vi "Read Data from Caller.vi"(7 "lv_icon.vi":refnum<vi>, 8 "error in":errorcluster, 10 "Default body text":T1 {"Body Text Spec"."Alignment" items=["left", "center", "right"]}, 11 "Init? (F)":bool) -> (0 "error out":errorcluster, 1 "Library Icon":picture, 2 "Icon Editor Invoker Type":T5, 3 "data":T4={"Text Visible?"=FALSE, "Text Opacity"=0, "Templ Visible?"=FALSE, "Templ Opacity"=0, "Relative Path from 1 to 2"=path "", "Image"=bytes[0], "All User Layers"=[], "Body Text"={"Line 1 text"="", "Line 2 text"="", "Line 3 text"="", "Line 4 text"="", "Line 1 color"=0, "Line 2 color"=0, "Line 3 color"=0, "Line 4 color"=0, "Body Text Spec"={"Font"="", "Alignment"=0, "Size"=3}, "Center text vertically"=FALSE, "Capitalize Text"=FALSE}} {"Body Text"."Body Text Spec"."Alignment" items=["left", "center", "right"]}, 4 "Valid?":bool, 5 "Valid Library icon?":bool)   [LabVIEW 2020]
uses:
  vi.lib/LabVIEW Icon API/lv_icon/Classes/Layer/Layer.lvclass
  <resource>/plugins/IconEditor/Icon Editor Invoker Type.ctl
  lv_icon.lvlib
  vi.lib/LabVIEW Icon API/lv_icon/Controls/LabVIEW Icon Stored Information.ctl
  vi.lib/LabVIEW Icon API/lv_icon/Controls/Font.ctl
  vi.lib/LabVIEW Icon API/lv_icon/Controls/Alignment.ctl
  vi.lib/LabVIEW Icon API/lv_icon/Controls/BodyText.ctl
panel:
  in  "String":string="Palette Icon"
  in  "Localized string":string="Icon Editor"
  # "Localized Strings"
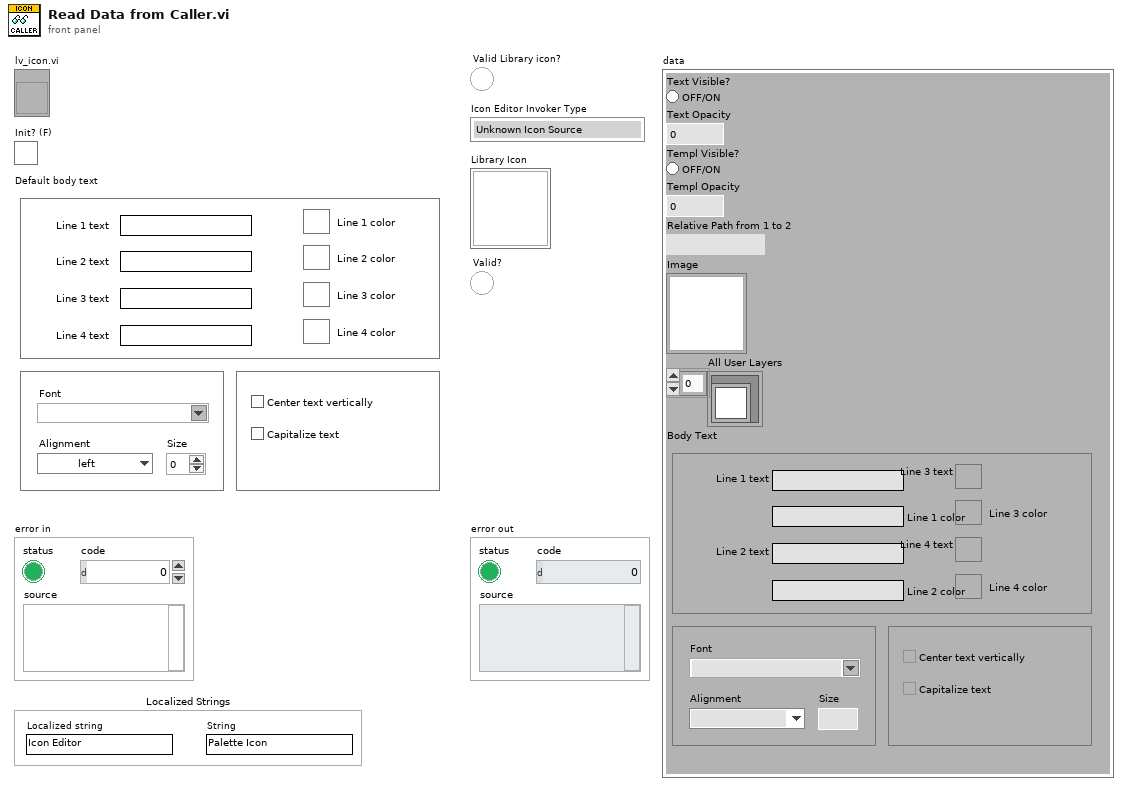
[diagram p1: front panel]
types:
  T1 = typedef "BodyText.ctl" = cluster{"Line 1 text":string, "Line 2 text":string, "Line 3 text":string, "Line 4 text":string, "Line 1 color":u32, "Line 2 color":u32, "Line 3 color":u32, "Line 4 color":u32, "Body Text Spec":cluster{"Font":T2, "Alignment":T3, "Size":u8}, "Center text vertically":bool, "Capitalize Text":bool}
  T2 = typedef "Font.ctl" = string
  T3 = typedef "Alignment.ctl" = u16
  T4 = typedef "LabVIEW Icon Stored Information.ctl" = cluster{"Text Visible?":bool, "Text Opacity":u8, "Templ Visible?":bool, "Templ Opacity":u8, "Relative Path from 1 to 2":path, "Image":picture, "All User Layers":refnum<class "Layer.lvclass">[], "Body Text":T1}
  T5 = typedef "Icon Editor Invoker Type.ctl" = enum32{"Unknown Icon Source", "VI Icon", "Library Icon (any library type)", "Palette icon", "Icon from App Method"}
  T6 = typedef "Who Invoked Icon Editor.ctl" = cluster{"Icon Editor Invoker Type":T5, "App Refnum of Invoker":refnum<vi>, "Qualified Name of Invoker":string, "Path to Invoker":path}
  T7 = typedef "imagedata.ctl" = cluster{"image type":i32, "image depth":i32, "image":u8[], "mask":u8[], "colors":u32[], "Rectangle":cluster{"left":i16, "top":i16, "right":i16, "bottom":i16}}
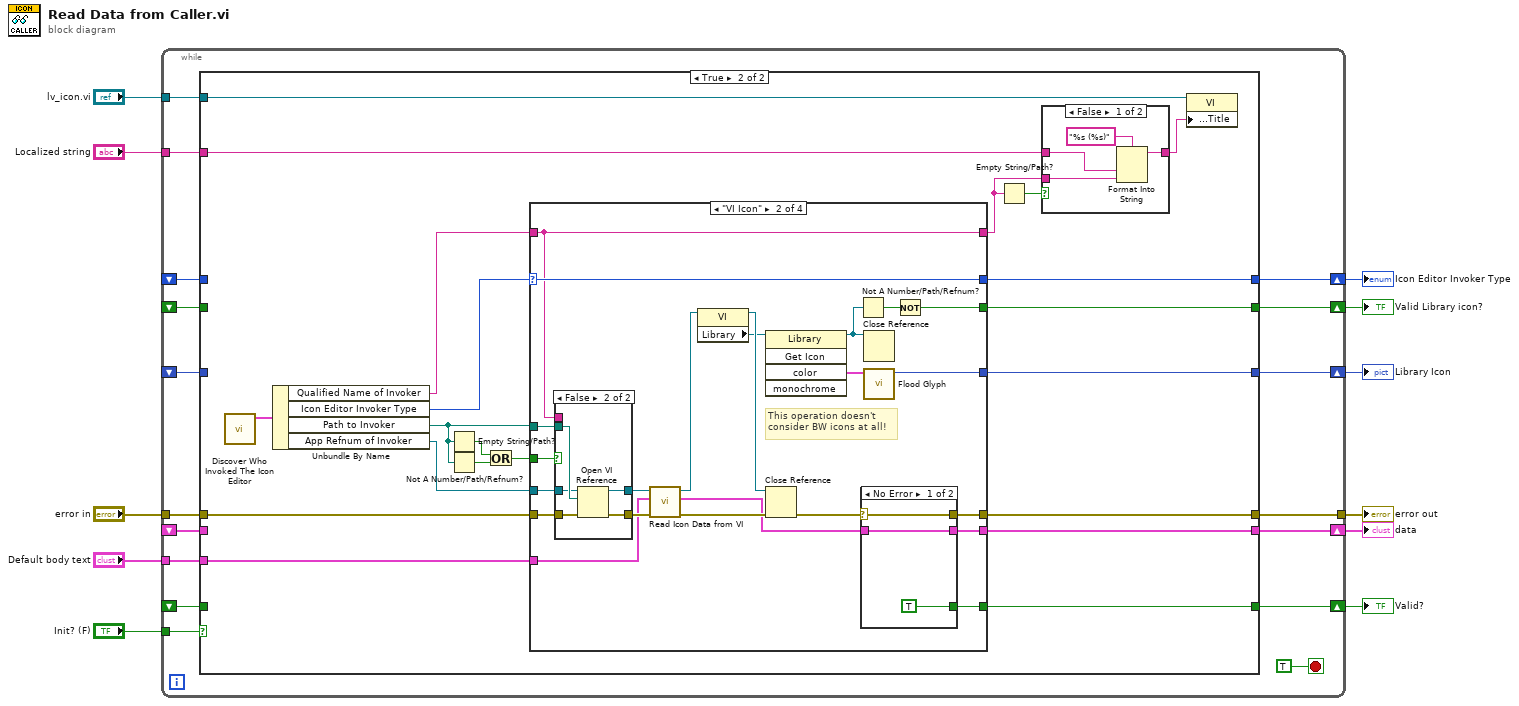
[diagram p0: block diagram]
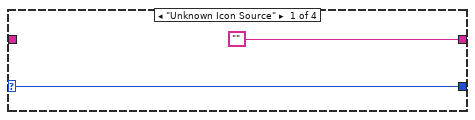
[diagram p4: hidden frame]
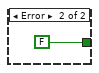
[diagram p5: hidden frame]
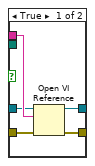
[diagram p6: hidden frame]
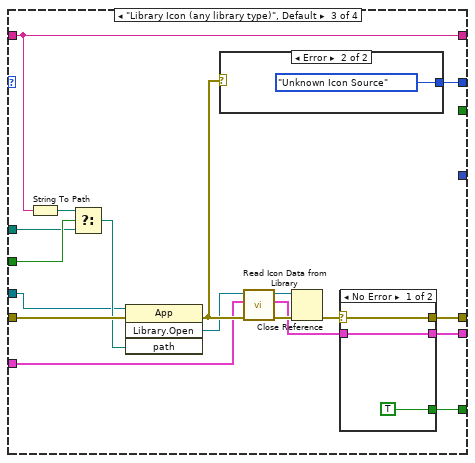
[diagram p7: hidden frame]
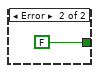
[diagram p8: hidden frame]
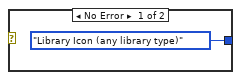
[diagram p9: hidden frame]
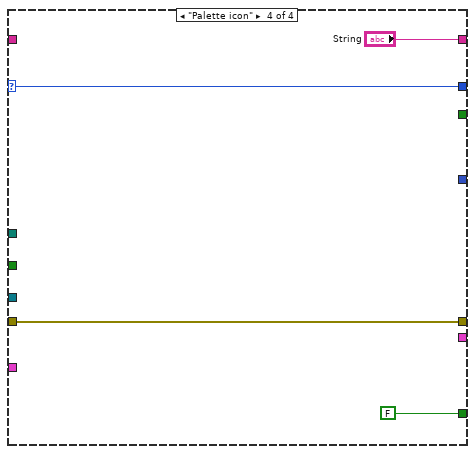
[diagram p10: hidden frame]
diagram:
  n1 = while {
    tunnel: [w28] -> w10
    tunnel: "error in" -> [w27]
    tunnel: "Init? (F)" -> [w24]
    tunnel: "lv_icon.vi" -> [w22]
    shift-right: [w23] -> w7
    shift-left: _ -> [w19]
    shift-right: [w25] -> w5
    shift-left: _ -> [w20]
    shift-right: [w26] -> w6
    shift-left: _ -> [w18]
    shift-right: [w17] -> w4
    shift-left: _ -> [w16]
    shift-right: [w15] -> w3
    shift-left: _ -> [w14]
    tunnel: "Default body text" -> [w13]
    tunnel: "Localized string" -> [w12]
    stop <- TRUE stop-if-true
    n2 = case shown="True" w24 {
      tunnel: [w34 w55] -> w28
      tunnel: [w33 w53] -> w25
      tunnel: [w31 w52] -> w26
      tunnel: w27 -> [w34 w54]
      tunnel: [w32 w48] -> w23
      tunnel: w22 -> [_ w39]
      tunnel: w20 -> [w33 _]
      tunnel: w19 -> [w32 _]
      tunnel: w18 -> [w31 _]
      tunnel: [w30 w42] -> w17
      tunnel: w16 -> [w30 _]
      tunnel: [w29 w35] -> w15
      tunnel: w14 -> [w29 _]
      tunnel: w13 -> [_ w41]
      tunnel: w12 -> [_ w40]
      frame False {
      }
      frame True {
        n3 = call <resource>:"Discover Who Invoked The Icon Editor.vi"() -> ("Who Invoked The Icon Editor?"=w51:T6)  [unwired: 11 out]
        n4 = Unbundle By Name(w51) -> ("Qualified Name of Invoker"=w44:string, "Icon Editor Invoker Type"=w49:T5, "Path to Invoker"=w43:path, "App Refnum of Invoker"=w50:refnum<vi>)
        n5 = Empty String/Path?(string/path=w43) -> (empty?=w47:bool)
        n6 = Not A Number/Path/Refnum?(number/path/refnum=w43) -> (NaN/Path/Refnum?=w46:bool)
        n7 = Or(x=w47, y=w46) -> (x .or. y?=w45:bool)
        n8 = case shown="\"VI Icon\"" w49 {
          selector: w49 -> [w62 w78 _ w125]
          tunnel: [_ w82 w114 w127] -> w55
          tunnel: [_ w65 w100 _] -> w53
          tunnel: [_ w63 w101 FALSE] -> w52
          tunnel: w54 -> [_ w84 w117 w127]
          tunnel: w50 -> [_ w79 w109 _]
          tunnel: [w62 w78 w108 w125] -> w48
          tunnel: w44 -> [_ w66 w103 _]
          tunnel: w43 -> [_ w76 w106 _]
          tunnel: w45 -> [_ w77 w107 _]
          tunnel: [_ w71 _ _] -> w42
          tunnel: [_ w68 _ _] -> w35
          tunnel: w41 -> [_ w67 w104 _]
          tunnel: ["" w66 w103 "String"] -> w36
          frame "Unknown Icon Source" {
          }
          frame "VI Icon" {
            # "This operation doesn't\nconsider BW icons at all!"
            n9 = case shown="False" w77 {
              tunnel: [w92 w96] -> w80
              tunnel: [w94 w99] -> w85
              tunnel: w84 -> [w93 w98]
              tunnel: w79 -> [w90 w95]
              tunnel: w66 -> [w91 _]
              tunnel: w76 -> [_ w97]
              frame True {
                n10 = Open VI Reference(application reference (local)=w90, vi path=w91, error in (no error)=w93) -> (vi reference=w92:refnum<vi>, error out=w94:errorcluster)  [unwired: 3 out]
              }
              frame False {
                n11 = Open VI Reference(application reference (local)=w95, vi path=w97, error in (no error)=w98) -> (vi reference=w96:refnum<vi>, error out=w99:errorcluster)  [unwired: 3 out]
              }
            }
            n12 = call "Read Icon Data from VI.vi"("error in (no error)"=w85, "Default body text"=w67, "VI Ref in"=w80) -> ("error out"=w83:errorcluster, "Data"=w64:T4, "VI Ref out"=w74:refnum<vi>)  [unwired: 6 in]
            n13 = property class="VI"(reference=w74) -> (reference out=w75:refnum<vi>, "Library"=w73:refnum<vi>)  [unwired: 1 in, 1 out]
            n14 = invoke class="Library" method="Get Icon"(reference=w73) -> (reference out=w70:refnum<vi>, "color"=w72:T7)  [unwired: 4 in, 3 out]
            n15 = Close Reference(reference=w75, error in (no error)=w83) -> (error out=w81:errorcluster)
            n16 = Not A Number/Path/Refnum?(number/path/refnum=w70) -> (NaN/Path/Refnum?=w69:bool)
            n17 = case shown="No Error" w81 {
              selector: w81 -> [w88 _]
              tunnel: [w88 _] -> w82
              tunnel: [w86 _] -> w65
              tunnel: [TRUE FALSE] -> w63
              tunnel: w64 -> [w86 _]
              frame No Error {
              }
              frame Error {
              }
            }
            n18 = Close Reference(reference=w70) -> ()  [unwired: 1 in, 1 out]
            n19 = call "Flood Glyph.vi"("image data"=w72) -> ("Pic Out"=w71:picture)  [unwired: 1 in, 9 out]
            n20 = Not(x=w69) -> (.not. x?=w68:bool)
          }
          frame "Library Icon (any library type)", Default {
            n21 = String To Path(string=w103) -> (path=w105:path)
            n22 = Select(t=w105, s=w107, f=w106) -> (s? t:f=w112:path)
            n23 = invoke class="App" method="Library.Open"(reference=w109, error in=w117, "path"=w112) -> (error out=w115:errorcluster, "Open Library"=w111:refnum<vi>)  [unwired: 1 in, 2 out]
            n24 = case shown="Error" w115 {
              tunnel: [Icon_Editor_Invoker_Type."Library Icon (any library type)" ("Icon Editor Invoker Type") Icon_Editor_Invoker_Type."Unknown Icon Source" ("Icon Editor Invoker Type")] -> w108
              frame No Error {
              }
              frame Error {
              }
            }
            n25 = call "Read Icon Data from Library.vi"("error in"=w115, "Default body text"=w104, "Library in"=w111) -> ("error out"=w116:errorcluster, "Data"=w102:T4, "Library out"=w110:refnum<vi>)  [unwired: 6 in]
            n26 = Close Reference(reference=w110, error in (no error)=w116) -> (error out=w113:errorcluster)
            n27 = case shown="No Error" w113 {
              selector: w113 -> [w120 _]
              tunnel: [w120 _] -> w114
              tunnel: [w118 _] -> w100
              tunnel: [TRUE FALSE] -> w101
              tunnel: w102 -> [w118 _]
              frame No Error {
              }
              frame Error {
              }
            }
          }
          frame "Palette icon" {
          }
        }
        n28 = Empty String/Path?(string/path=w36) -> (empty?=w37:bool)
        n29 = case shown="False" w37 {
          tunnel: w40 -> [w59 w60]
          tunnel: w36 -> [w57 _]
          tunnel: [w56 w60] -> w38
          frame False {
            n30 = Format Into String(format string="%s (%s)", w59, w57) -> (resulting string=w56:string)  [unwired: 2 in, 1 out]
          }
          frame True {
          }
        }
        n31 = property class="VI"(reference=w39, "Front Panel.Title"=w38) -> ()  [unwired: 1 in, 2 out]
      }
    }
  }
  "Valid?" <- w6
  "Icon Editor Invoker Type" <- w7
  "data" <- w5
  "Library Icon" <- w4
  "Valid Library icon?" <- w3
  "error out" <- w10
